vi "hamming top.vi"() -> ()   [LabVIEW 2025]
uses:
  <vilib>/numeric/Random Number (Range) U64.vi
panel:
  in  "error selector":u16(ring) items=["no error", "single bit error", "double bit error"]
  out "decoded sentence":string
  in  "input sentence":string
  out "message - U8 boolean":bool[](array[boolean])
  out "transmitted message":bool[](array[boolean])
  in  "number of control bits":i32
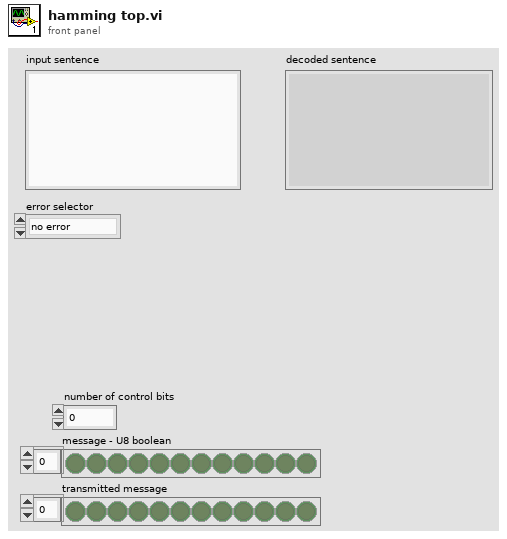
[diagram p1: front panel]
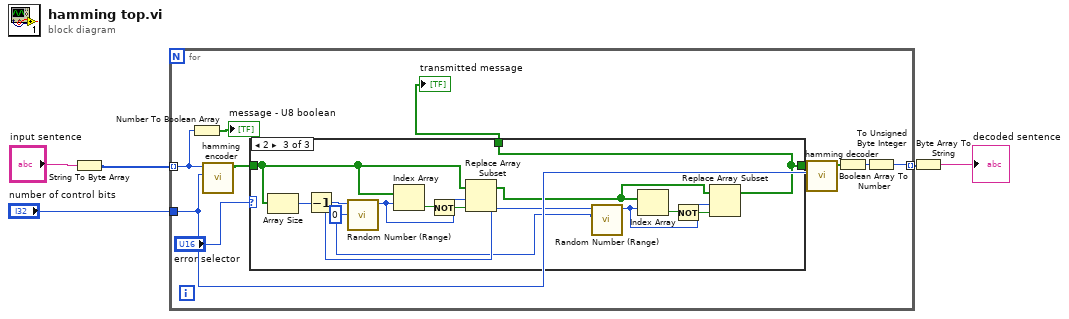
[diagram p0: block diagram]
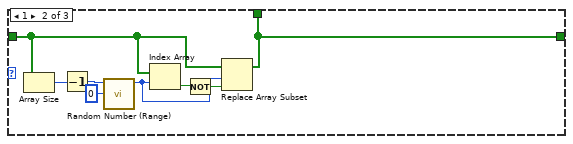
[diagram p3: hidden frame]
diagram:
  n1 = String To Byte Array(string="input sentence") -> (unsigned byte array=w2:u8[])
  n2 = for {
    tunnel: "number of control bits" -> [w15]
    tunnel: w2 -> [w13] mode=indexing
    tunnel: [w10] -> w1 mode=indexing
    n3 = Number To Boolean Array(number=w13) -> (Boolean array=→"message - U8 boolean":bool[])
    n4 = call "hamming encoder.vi"("number of control bits"=w15, "message"=w13) -> ("output array"=w7:bool[])  [unwired: 9 in]
    n5 = case shown="2" "error selector" {
      tunnel: [w16 w18 w25] -> w8
      tunnel: w7 -> [w16 w17 w27]
      tunnel: [w16 w18 w25] -> w6
      frame 0, Default {
      }
      frame 1 {
        n6 = Array Size(array=w17) -> (size(s)=w23:i32)
        n7 = Decrement(x=w23) -> (x-1=w24:i32)
        n8 = call-poly <vilib>:"Random Number (Range).vi"("lower bound (0)"=u64 0, "upper bound (100)"=w24) -> ("number"=w20:u64)  [unwired: 9 in]
        n9 = Index Array(array=w17, index=w20) -> (element=w21:bool)
        n10 = Not(x=w21) -> (.not. x?=w19:bool)
        n11 = Replace Array Subset(array=w17, new element=w19, index=w20) -> (w18:bool[])
      }
      frame 2 {
        w28 = u64 0 ("lower bound (0)")
        n12 = Array Size(array=w27) -> (size(s)=w36:i32)
        n13 = Decrement(x=w36) -> (x-1=w29:i32)
        n14 = call-poly <vilib>:"Random Number (Range).vi"("lower bound (0)"=w28, "upper bound (100)"=w29) -> ("number"=w34:u64)  [unwired: 9 in]
        n15 = Index Array(array=w27, index=w34) -> (element=w35:bool)
        n16 = Not(x=w35) -> (.not. x?=w33:bool)
        n17 = Replace Array Subset(array=w27, new element=w33, index=w34) -> (w26:bool[])
        n18 = call-poly <vilib>:"Random Number (Range).vi"("lower bound (0)"=w28, "upper bound (100)"=w29) -> ("number"=w31:u64)  [unwired: 9 in]
        n19 = Index Array(array=w26, index=w31) -> (element=w32:bool)
        n20 = Not(x=w32) -> (.not. x?=w30:bool)
        n21 = Replace Array Subset(array=w26, new element=w30, index=w31) -> (w25:bool[])
      }
    }
    "transmitted message" <- w6
    n22 = call "hamming decoder.vi"("number of control bits"=w15, "Encoded Message"=w8) -> ("decoded message"=w12:bool[])  [unwired: 9 in]
    n23 = Boolean Array To Number(Boolean array=w12) -> (number=w11:u32)
    n24 = To Unsigned Byte Integer(number=w11) -> (unsigned 8bit integer=w10:u8)
  }
  n25 = Byte Array To String(unsigned byte array=w1) -> (string=→"decoded sentence":string)
